vi "Q15_Channel_Pick.vi"() -> ()   [LabVIEW 2018]
doc: "Use this template to build a VI to use as a subVI."
panel:
  out "D":dbl[](array[numeric])
  out "C":dbl[](array[numeric])
  out "B":dbl
  out "A":dbl[](array[numeric])
  in  "Data":dbl[][](array[numeric])
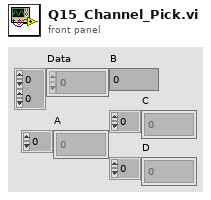
[diagram p1: front panel]
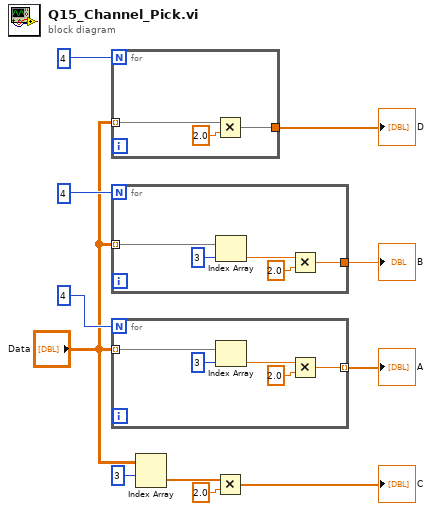
[diagram p0: block diagram]
diagram:
  n1 = for {
    N: 4 -> [_]
    tunnel: "Data" -> [w13] mode=indexing
    tunnel: [w12] -> w1
    n2 = Multiply(x=w13, y=2.0) -> (x*y=w12:dbl[])
  }
  "D" <- w1
  n3 = for {
    N: 4 -> [_]
    tunnel: "Data" -> [w18] mode=indexing
    tunnel: [w15] -> w8
    n4 = Index Array(array=w18, index=3) -> (element=w16:dbl)
    n5 = Multiply(x=w16, y=2.0) -> (x*y=w15:dbl)
  }
  "B" <- w8
  n6 = for {
    N: 4 -> [_]
    tunnel: "Data" -> [w23] mode=indexing
    tunnel: [w20] -> w10 mode=indexing
    n7 = Index Array(array=w23, index=3) -> (element=w21:dbl)
    n8 = Multiply(x=w21, y=2.0) -> (x*y=w20:dbl)
  }
  "A" <- w10
  n9 = Index Array(array="Data", index (row)=3) -> (element=w5:dbl[])  [unwired: 1 in]
  n10 = Multiply(x=w5, y=2.0) -> (x*y=→"C":dbl[])
